vi "create.request.vi"(8 "error in":errorcluster, 9 "Assets":string[](array[string]), 10 "Start Time":timestamp format="%<%x %.3X>T", 11 "Title":string) -> (0 "error out":errorcluster, 1 "Request":string)   [LabVIEW 2020, in "Run.lvclass"]
uses:
  Run.lvclass
  <vilib>/JDP Science/JSONtext/Variant to JSON Text.vi
  <vilib>/JDP Science/JSONtext/LVClass Serializer/JSONtext LVClass Serializer.lvclass
  Run.lvclass/Run.ctl
  2fbe8fca-b16e-45d9-9acc-ed174a081b12.vi
  21ec94b3-9936-4974-8d50-7fe96fbbf006.vi
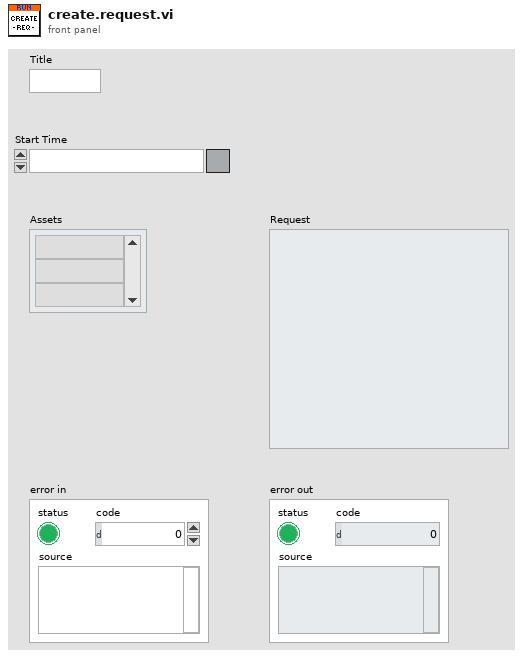
[diagram p1: front panel]
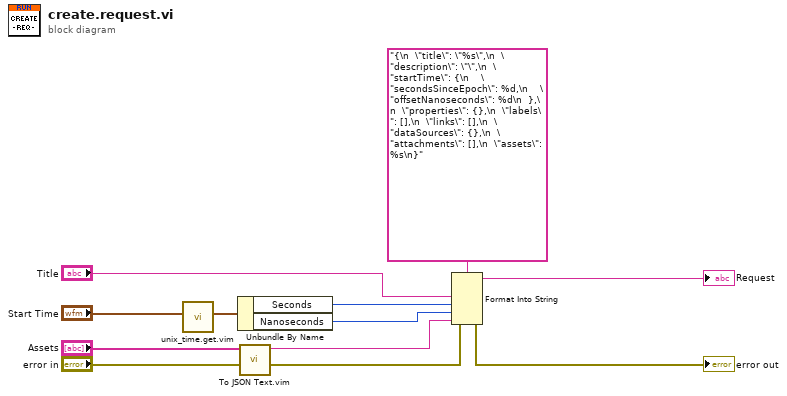
[diagram p0: block diagram]
diagram:
  n1 = call "unix_time.get.vim"("Time Stamp (empty: now) [single or array]"="Start Time") -> ("UNIX Timestamp"=w6:cluster{"Seconds":i64, "Nanoseconds":i64})  [unwired: 10 in]
  n2 = Unbundle By Name(w6) -> ("Seconds"=w3:i64, "Nanoseconds"=w4:i64)
  n3 = call "To JSON Text.vim"("error in (no error)"="error in", "Anything"="Assets") -> ("error out"=w2:errorcluster, "<JSON>"=w1:string)  [unwired: 8 in]
  n4 = Format Into String(format string="{\n  \"title\": \"%s\",\n  \"description\": \"\",\n  \"startTime\": {\n    \"secondsSinceEpoch\": %d,\n    \"offsetNanoseconds\": %d\n  },\n  \"properties\": {},\n  \"labels\": [],\n  \"links\": [],\n  \"dataSources\": {},\n  \"attachments\": [],\n  \"assets\": %s\n}", error in=w2, "Title", w3, w4, w1) -> (resulting string=→"Request":string, error out=→"error out":errorcluster)  [unwired: 1 in]
